vi "Condition_Check_Quality.vi"(8 "error in (no error)":errorcluster={"status"=FALSE, "code"=0, "source"="\"\""}, 10 "max age":string, 11 "ParameterValue":string) -> (0 "error out":errorcluster={"status"=FALSE, "code"=0, "source"="\"\""}, 2 "status ok":bool, 3 "Valid/stale/invalid state":string)   [LabVIEW 2026]
doc: "INTENT: Verify signal freshness. LOGIC: Reject impossible timestamps, age beyond limit and sensor invalid flags."
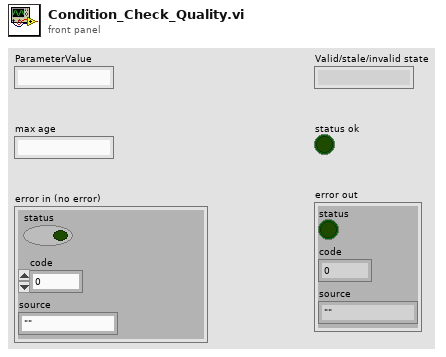
[diagram p1: front panel]
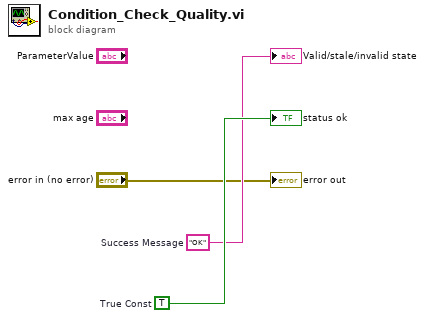
[diagram p0: block diagram]
diagram:
  w3 = TRUE  # True Const
  w2 = "OK"  # Success Message
  "Valid/stale/invalid state" <- w2
  "status ok" <- w3
  "error out" <- "error in (no error)"
